vi "Read GWS File.vi"(11 "Path":path=path "D:/同步空间/曲线生成/原始曲线/4、广五所 温冲箱--dfg.xls") -> (3 "Data Series":T1[](array[typedef]))   [LabVIEW 2020, in "Data Viewer.lvlib"]
uses:
  Data Viewer.lvlib
  Data Serie--cluster.ctl
  File Type--enum.ctl
  <vilib>/Utility/file.llb/Read Delimited Spreadsheet (string).vi
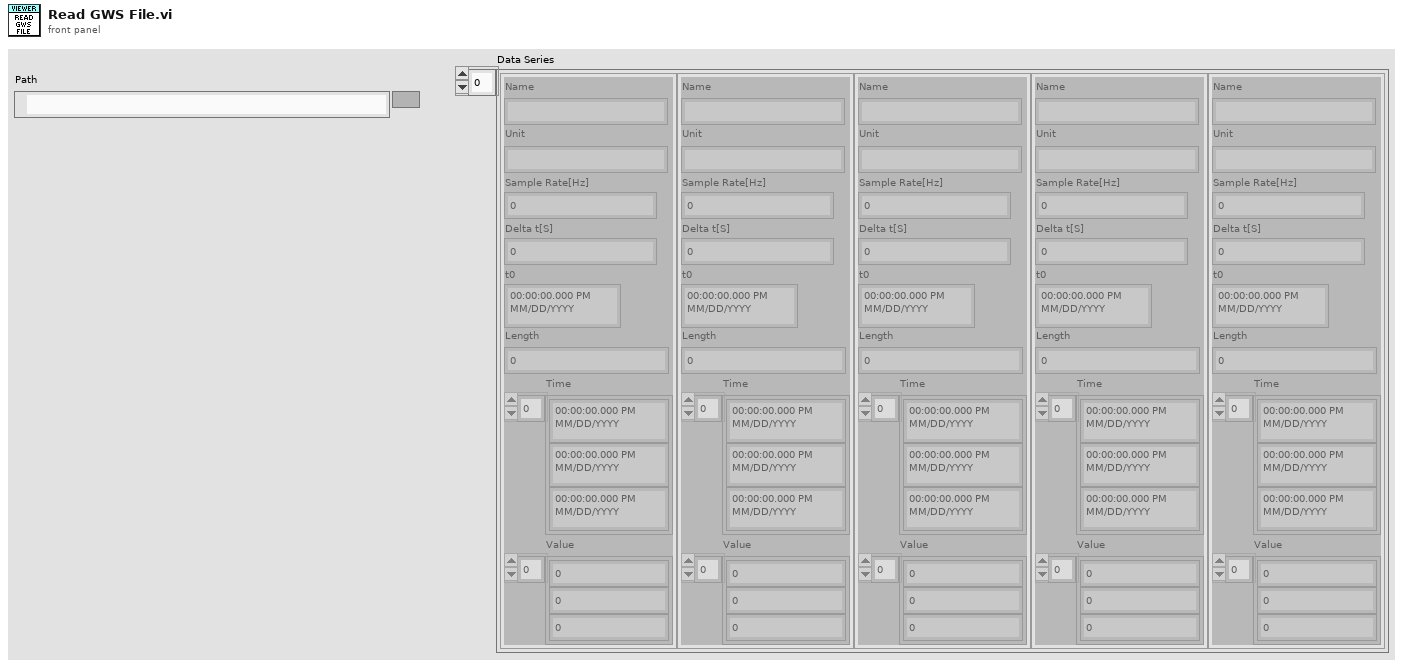
[diagram p1: front panel]
types:
  T1 = typedef "Data Viewer.lvlib/Data Serie--cluster.ctl" = cluster{"Name":string, "Unit":string, "Sample Rate[Hz]":dbl, "Delta t[S]":dbl, "t0":timestamp, "Length":i32, "Time":timestamp[], "Value":dbl[]}
  T2 = typedef "Data Viewer.lvlib/File Type--enum.ctl" = enum16{"伟思环境箱", "增达环境箱", "广五所环境箱", "无纸记录仪", "帕捷SA00339", "记录仪840", "记录仪8400", "记录仪MR888", "*.csv"}
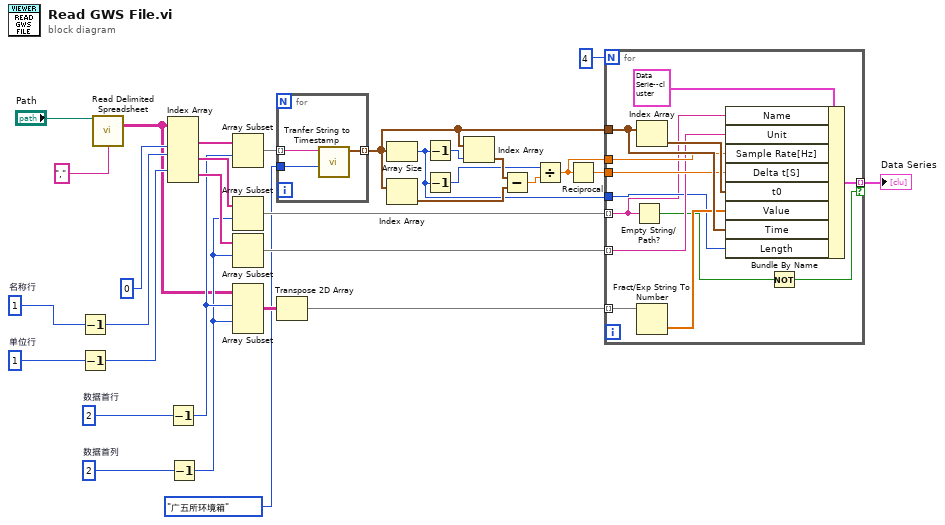
[diagram p0: block diagram]
diagram:
  w25 = 2  # 数据首列
  w26 = 2  # 数据首行
  w28 = 1  # 单位行
  w30 = 1  # 名称行
  n1 = Decrement(x=w30) -> (x-1=w21:i32)
  n2 = Decrement(x=w28) -> (x-1=w20:i32)
  n3 = call-poly <vilib>:"Read Delimited Spreadsheet.vi"("file path (dialog if empty)"="Path", "delimiter (\\t)"="," ("delimiter (\\t)")) -> ("all rows"=w2:string[][])  [unwired: 8 in, 5 out]
  n4 = Index Array(array=w2, index (col) #1=0 ("disabled index (col)"), index (row) #2=w21, index (row) #3=w20) -> (element #1=w31:string[], element #2=w29:string[], element #3=w27:string[])  [unwired: 3 in]
  n5 = Decrement(x=w26) -> (x-1=w19:i32)
  n6 = Decrement(x=w25) -> (x-1=w18:i32)
  n7 = Array Subset(array=w31, index=w19) -> (w9:string[])  [unwired: 1 in]
  n8 = Array Subset(array=w29, index=w18) -> (w23:string[])  [unwired: 1 in]
  n9 = Array Subset(array=w27, index=w18) -> (w22:string[])  [unwired: 1 in]
  n10 = Array Subset(array=w2, index (row)=w19, index (col)=w18) -> (w24:string[][])  [unwired: 2 in]
  n11 = for {
    tunnel: [w35] -> w8 mode=indexing
    tunnel: w9 -> [w34] mode=indexing
    tunnel: File_Type--enum."广五所环境箱" ("File Type") -> [w33]
    n12 = call "Tranfer String to Timestamp.vi"("File Type"=w33, "String"=w34) -> ("time stamp"=w35:timestamp)  [unwired: 9 in]
  }
  n13 = Transpose 2D Array(2D array=w24) -> (transposed array=w17:string[][])
  n14 = Array Size(array=w8) -> (size(s)=w4:i32)
  n15 = Index Array(array=w8) -> (element=w14:timestamp)  [unwired: 1 in]
  n16 = Decrement(x=w4) -> (x-1=w16:i32)
  n17 = Decrement(x=w4) -> (x-1=w6:i32)
  n18 = Index Array(array=w8, index=w16) -> (element=w15:timestamp)
  n19 = Subtract(x=w15, y=w14) -> (x-y=w13:dbl)
  n20 = Divide(x=w6, y=w13) -> (x/y=w12:dbl)
  n21 = Reciprocal(x=w12) -> (1/x=w11:dbl)
  n22 = for {
    N: 4 -> [_]
    tunnel: w23 -> [w37] mode=indexing
    tunnel: w22 -> [w40] mode=indexing
    tunnel: w17 -> [w45] mode=indexing
    tunnel: w8 -> [w46]
    tunnel: w12 -> [w43]
    tunnel: w11 -> [w42]
    tunnel: [w41] -> w10 mode=indexing if=w36
    tunnel: w4 -> [w39]
    n23 = Empty String/Path?(string/path=w37) -> (empty?=w38:bool)
    n24 = Index Array(array=w46) -> (element=w47:timestamp)  [unwired: 1 in]
    n25 = Fract/Exp String To Number(string=w45) -> (number=w44:dbl[])  [unwired: 3 in, 1 out]
    n26 = Bundle By Name(cluster=T1 {"Name"="", "Unit"="", "Sample Rate[Hz]"=0.0, "Delta t[S]"=0.0, "t0"=timestamp(0 s since 1904-01-01), "Length"=0, "Time"=[], "Value"=[]} ("Data Serie"), "Name"=w37, "Unit"=w40, "Sample Rate[Hz]"=w43, "Delta t[S]"=w42, "t0"=w47, "Value"=w44, "Time"=w46, "Length"=w39) -> (w41:T1)
    n27 = Not(x=w38) -> (.not. x?=w36:bool)
  }
  "Data Series" <- w10
